vi "DAC Run.vi"(8 "error in":errorcluster, 11 "DAC HeatFlow AIV in":refnum<class "DAC HeatFlow AIV.lvclass">) -> (0 "error out":errorcluster, 3 "DAC HeatFlow AIV out":refnum<class "DAC HeatFlow AIV.lvclass">)   [LabVIEW 2019, in "DAC.lvlib" / "DAC HeatFlow AIV.lvclass"]
uses:
  DAC HeatFlow AIV.lvclass
  DAC.lvclass
  <vilib>/DAQmx/read.llb/DAQmx Read (Analog DBL 1Chan 1Samp).vi
  Results/Results Method.ctl
  Results/Results.lvlib
  Results/Heat Flow Results/Heat Flow Results.lvclass
  C:/Users/krio/Documents/LV_Projects/test-stand/App/DAC/DAC.lvclass
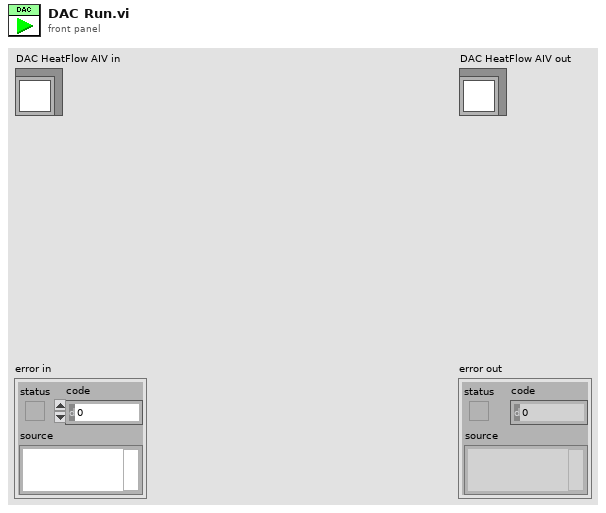
[diagram p1: front panel]
types:
  T1 = typedef "Results.lvlib/Results Method.ctl" = enum16{"Get", "Set"}
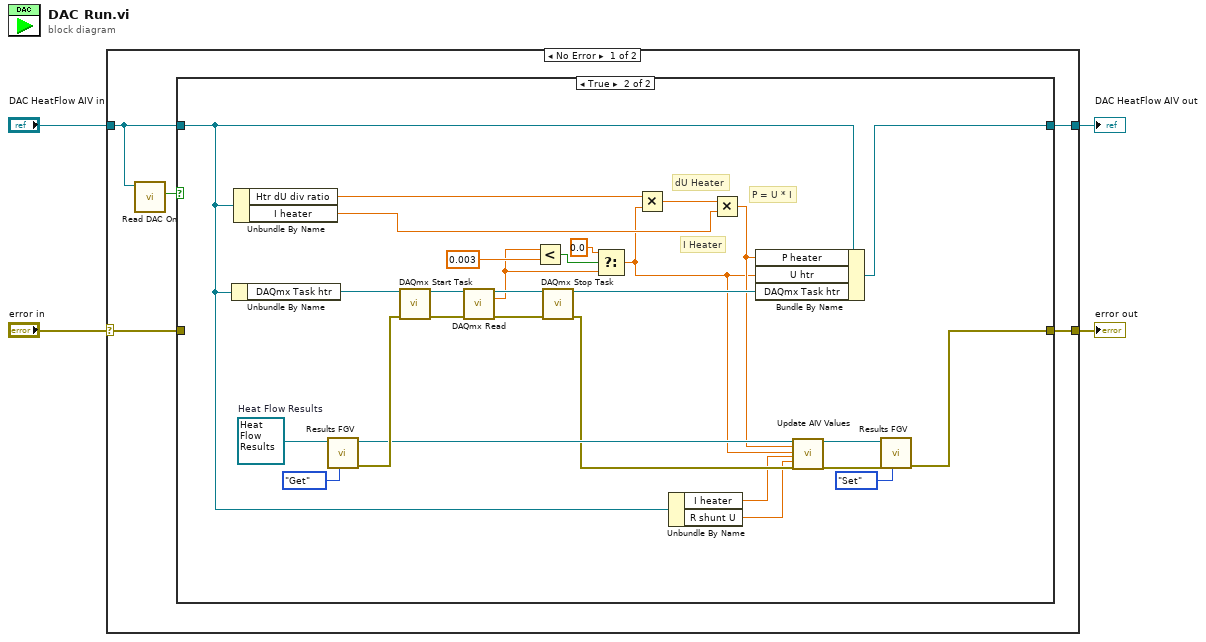
[diagram p0: block diagram]
diagram:
  n1 = case shown="No Error" "error in" {
    selector: "error in" -> [w7 w41]
    tunnel: [w6 w41] -> w2
    tunnel: [w8 w40] -> w1
    tunnel: "DAC HeatFlow AIV in" -> [w5 w40]
    frame No Error {
      n2 = call "Read DAC On.vi"("DAC in"=w5) -> ("DAC On"=w9:bool)  [unwired: 8 in, 2 out]
      n3 = case shown="True" w9 {
        tunnel: w5 -> [w11 w16]
        tunnel: [w11 w34] -> w8
        tunnel: w7 -> [w10 _]
        tunnel: [w10 w17] -> w6
        frame False {
        }
        frame True {
          w24 = refnum<class "Heat Flow Results.lvclass"> refnum  # Heat Flow Results
          # "I Heater"
          # "dU Heater"
          # "P = U * I"
          n4 = Unbundle By Name(w16) -> ("DAQmx Task htr"=w39:refnum<k21>)
          n5 = Unbundle By Name(w16) -> ("Htr dU div ratio"=w31:dbl, "I heater"=w30:dbl)
          n6 = call-dynamic "Results FGV.vi"("Method"=Results_Method."Get", "Results in"=w24) -> ("error out"=w23:errorcluster, "Results out"=w19:refnum<class "Heat Flow Results.lvclass">)  [unwired: 8 in]
          n7 = call <vilib>:"DAQmx Start Task.vi"("task/channels in"=w39, "error in"=w23) -> ("task out"=w38:refnum<k21>, "error out"=w36:errorcluster)  [unwired: 12 in]
          n8 = call-poly <vilib>:"DAQmx Read.vi"("task/channels in"=w38, "error in"=w36) -> ("task out"=w37:refnum<k21>, "data"=w26:dbl, "error out"=w35:errorcluster)  [unwired: 11 in]
          n9 = Less?(x=w26, y=0.003) -> (x < y?=w28:bool)
          n10 = call <vilib>:"DAQmx Stop Task.vi"("task/channels in"=w37, "error in"=w35) -> ("task out"=w33:refnum<k21>, "error out"=w18:errorcluster)  [unwired: 12 in]
          n11 = Select(t=0.0, s=w28, f=w26) -> (s? t:f=w12:dbl)
          n12 = Multiply(x=w31, y=w12) -> (x*y=w32:dbl)
          n13 = Unbundle By Name(w16) -> ("I heater"=w14:dbl, "R shunt U"=w15:dbl)
          n14 = Multiply(x=w32, y=w30) -> (x*y=w13:dbl)
          n15 = Bundle By Name(cluster=w16, "P heater"=w13, "U htr"=w12, "DAQmx Task htr"=w33) -> (w34:refnum<class "DAC HeatFlow AIV.lvclass">)
          n16 = call "Update AIV Values.vi"("Heat Flow Results in"=w19, "P_heater"=w13, "R htr dU"=w12, "I_heater"=w14, "R shunt U"=w15, "error in"=w18) -> ("Heat Flow Results out"=w21:refnum<class "Heat Flow Results.lvclass">, "error out"=w20:errorcluster)  [unwired: 12 in]
          n17 = call-dynamic "Results FGV.vi"("Method"=Results_Method."Set", "error in"=w20, "Results in"=w21) -> ("error out"=w17:errorcluster)  [unwired: 7 in, 1 out]
        }
      }
    }
    frame Error {
    }
  }
  "error out" <- w2
  "DAC HeatFlow AIV out" <- w1
